vi "configuration UI.vi"() -> ()   [LabVIEW 2013, in "alarms module editor node.lvclass"]
uses:
  alarms module editor node.lvclass
  <vilib>/NI/Configuration Framework/Node/NodeRef.ctl
  <vilib>/NI/Configuration Framework/Node/NISE_CEF_Node.lvclass
  <vilib>/NI/AMC/Message Queue.ctl
  <vilib>/NI/AMC/Message.ctl
  <vilib>/NI/Tools/Keyed Array/KeyedArray.ctl
  <vilib>/NI/Configuration Framework/Node/UserEventRef.ctl
  <vilib>/NI/Configuration Framework/Controls/EventCluster.ctl
  <vilib>/NI/Configuration Framework/Node/StopEvent.ctl
  <vilib>/NI/Configuration Framework/Node/RefreshUIEvent.ctl
  <vilib>/NI/Configuration Framework/Node/CacheState.ctl
  <vilib>/NI/Configuration Framework/Node/NodeChangeEvent.ctl
  module/configuration/boolean operation.ctl
  module/configuration/compare type.ctl
  <vilib>/NI/Tag Bus/tag/Data Type.ctl
  alarms module editor node.lvclass/alarms module editor node.ctl
  <vilib>/NI/Configuration Framework/serializable configuration/NISE_CEF_serializable configuration.lvclass/NISE_CEF_serializable configuration.ctl
  <vilib>/NI/Tag Bus/tag/tag descriptor.lvclass/tag descriptor.ctl
  <vilib>/NI/Module Execution Interface/Engine Configuration/engine configuration.lvclass/engine configuration.ctl
  <vilib>/Utility/LVClass/Get LV Class Name.vi
  <vilib>/NI/Configuration Framework/error generator/NISE_error generator.vi
  <vilib>/NI/Tag Bus Module Framework/channel/TBM channel.lvclass
  <vilib>/NI/Module Execution Interface/Engine Configuration/engine configuration.lvclass
  <vilib>/NI/DCAF/Tag Editor Core/Configuration Editor/Classes/Module editor node/module editor node.lvclass
  <vilib>/NI/DCAF/Tag Editor Core/Configuration Editor/Classes/Engine Parent/Engine Parent Editor Node.lvclass
  <vilib>/NI/Configuration Framework/serializable configuration/NISE_CEF_serializable configuration.lvclass
  module/configuration/alarms module configuration.lvclass
  <vilib>/NI/Tag Bus/tag/tag descriptor.lvclass
  <vilib>/NI/Tools/Keyed Array/Tools_KeyedArray.lvlib
  <vilib>/NI/AMC/AMC.lvlib
  <vilib>/NI/Configuration Framework/NISE_CEF_TreeControl.lvlib
panel:
  in  "node change":T1
  in  "cache state":T2
  in  "refresh UI":T3
  in  "stop event":T4
  in  "Tab Control":enum32{"Alarm Configuration", "Alarm Table"}(tab)
  in  "data type":T5
  in  "Limit":dbl
  in  "comparison op":T6
  in  "Input Tag":string(combo)
  in  "Unlatch Tag":string(combo)
  in  "Output Tag":string(combo)
  in  "Remove compare":bool
  in  "Add compare":bool
  in  "Comparisons list":i32(listbox)
  out "alarm name":string
  in  "Alarms":i32(listbox)
  in  "Remove alarm":bool
  in  "Add alarm":bool
  in  "operation":T7
  in  "Full Alarms Table":i32(listbox)
  in  "user event":T8
  in  "main queue":T9
  in  "node ref":T10
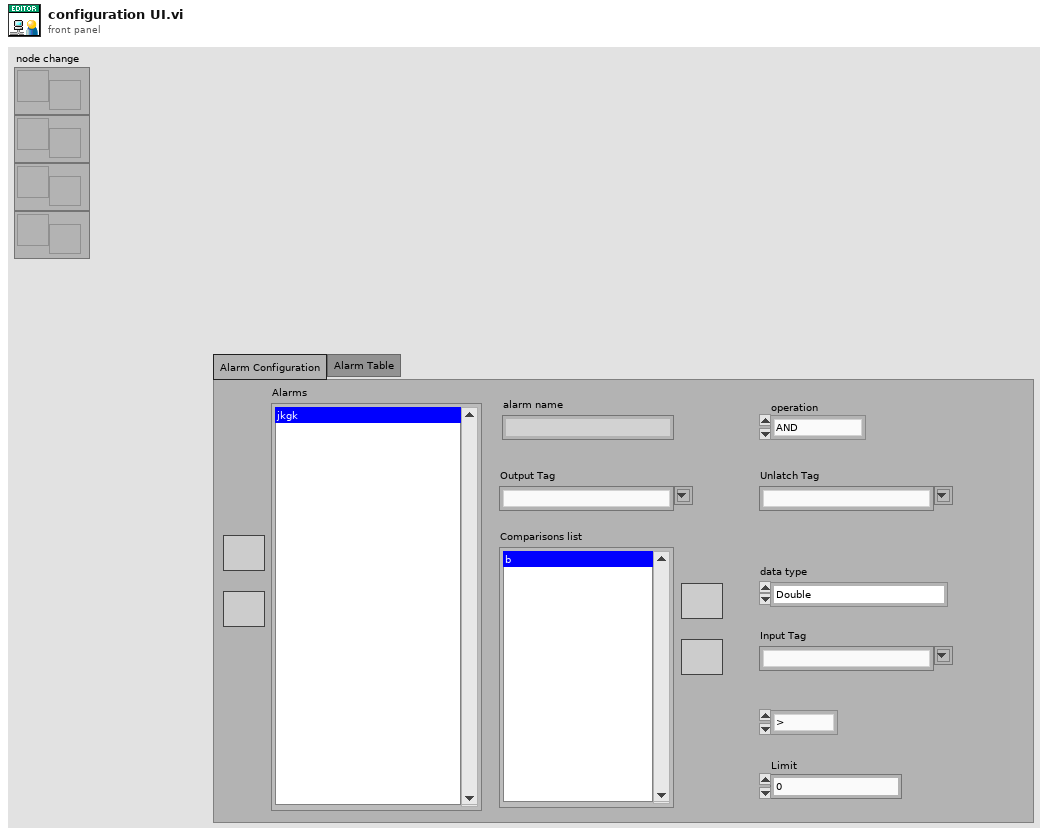
[diagram p1: front panel]
types:
  T1 = typedef "NISE_CEF_Node.lvclass/NodeChangeEvent.ctl" = refnum<user-event>
  T2 = typedef "NISE_CEF_Node.lvclass/CacheState.ctl" = refnum<user-event>
  T3 = typedef "NISE_CEF_Node.lvclass/RefreshUIEvent.ctl" = refnum<user-event>
  T4 = typedef "NISE_CEF_Node.lvclass/StopEvent.ctl" = refnum<user-event>
  T5 = typedef "tag bus.lvlib/tag descriptor.lvclass/Data Type.ctl" = enum16{"Double", "Single", "I64", "I32", "I16", "I8", "U64", "U32", "U16", "U8", "Boolean", "String", "Array of Double", "Array of Single", "Array of I64", "Array of I32", "Array of I16", "Array of I8", "Array of U64", "Array of U32", "Array of U16", "Array of U8", "Array of Boolean", "Array of String"}
  T6 = typedef "alarms module configuration.lvclass/compare type.ctl" = enum16{">", "<", ">=", "<=", "="}
  T7 = typedef "alarms module configuration.lvclass/boolean operation.ctl" = enum16{"AND", "OR"}
  T8 = typedef "NISE_CEF_Node.lvclass/UserEventRef.ctl" = refnum<user-event>
  T9 = typedef "AMC.lvlib/Message Queue.ctl" = refnum<queue>
  T10 = typedef "NISE_CEF_Node.lvclass/NodeRef.ctl" = refnum<data-value>
  T11 = enum8{"Enabled", "Disabled", "Disabled and Grayed Out"}
  T12 = typedef "alarms module configuration.lvclass/alarm configuration.ctl" = cluster{"alarm name":string, "comparisons":T13[], "unlatch":refnum<class "TBM channel.lvclass">, "output":refnum<class "TBM channel.lvclass">, "boolean op":T7}
  T13 = typedef "alarms module configuration.lvclass/alarm comparison.ctl" = cluster{"input channel":refnum<class "TBM channel.lvclass">, "limit":dbl, "comparison":T6}
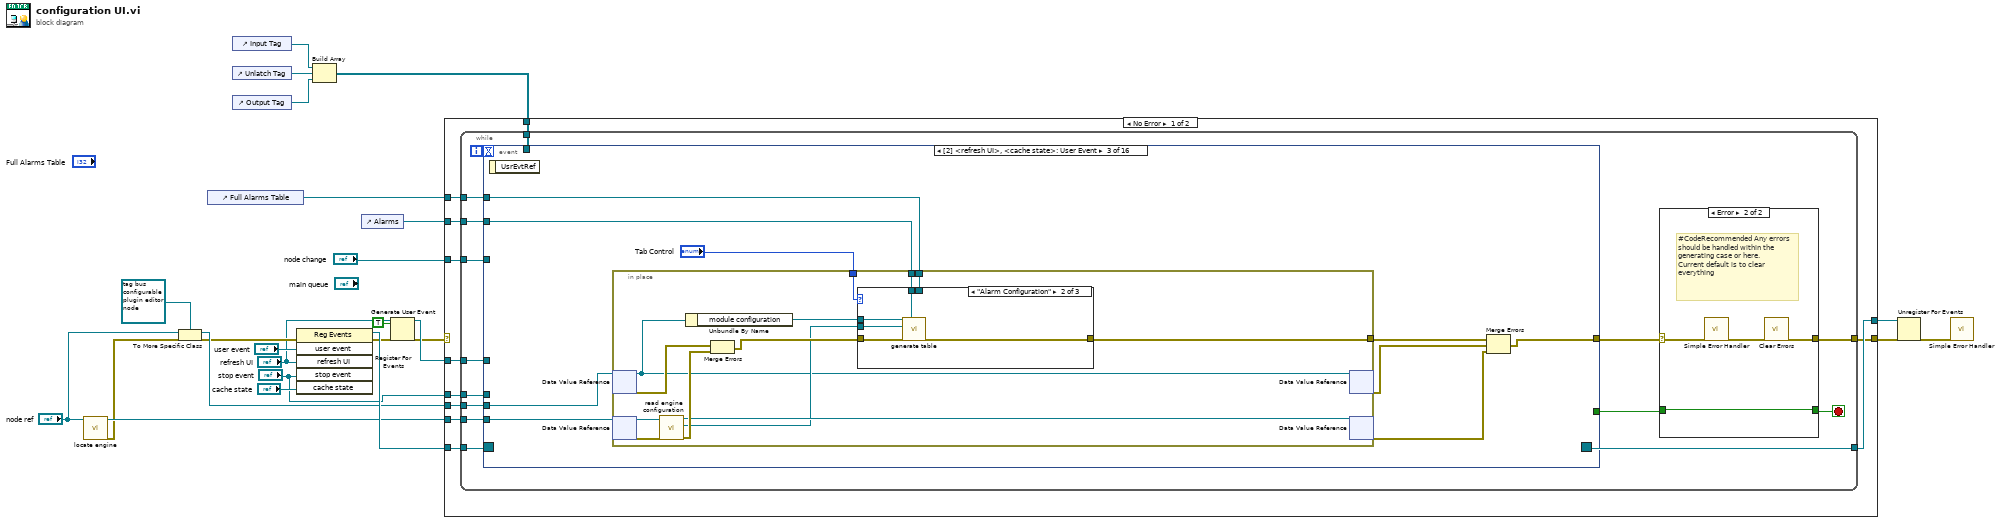
[diagram p0: block diagram]
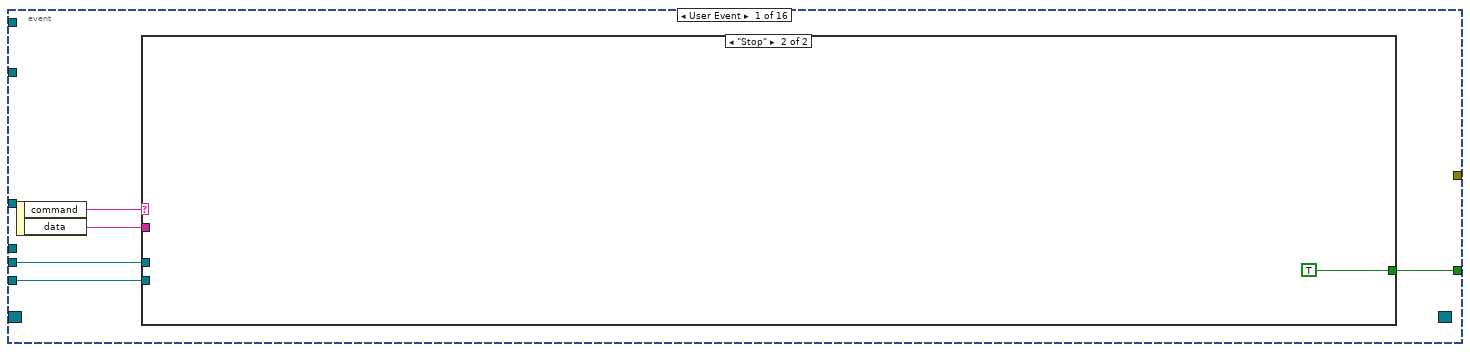
[diagram p3: hidden frame]
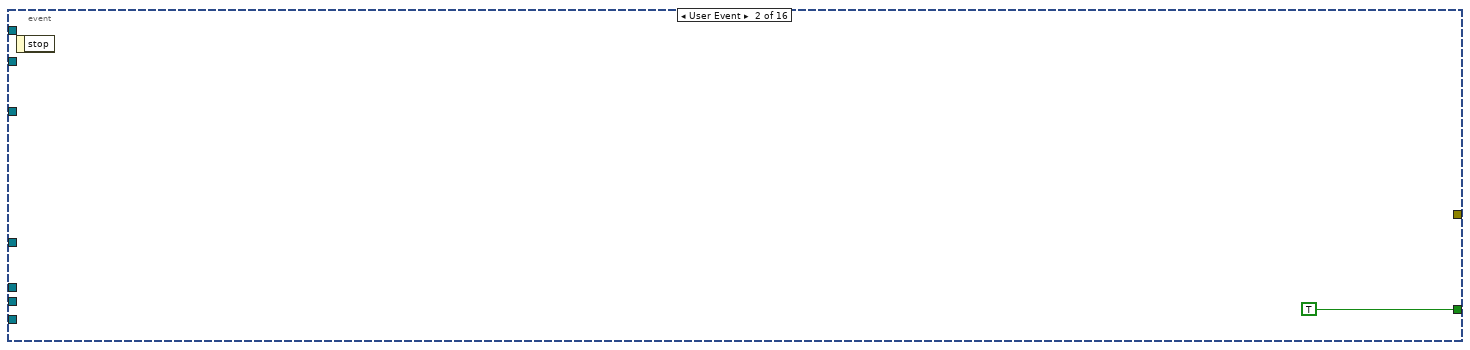
[diagram p5: hidden frame]
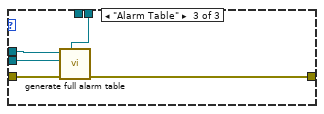
[diagram p7: hidden frame]
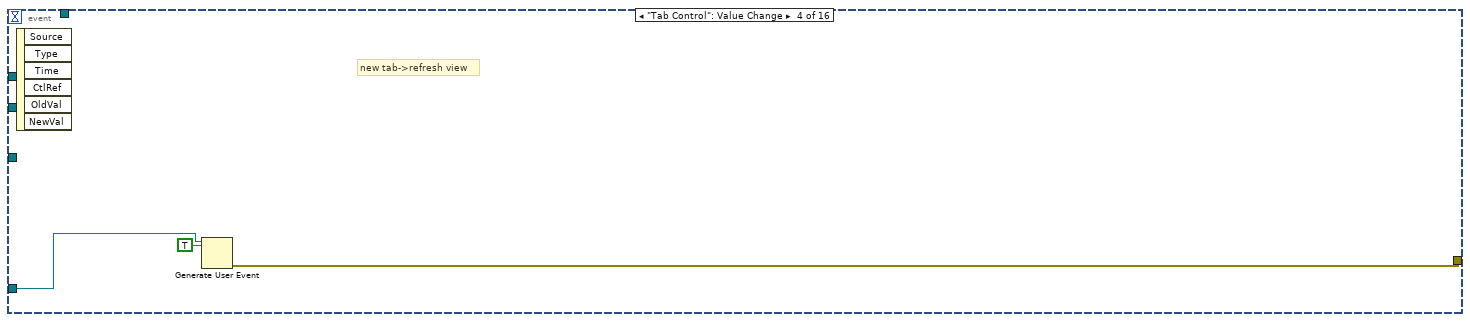
[diagram p8: hidden frame]
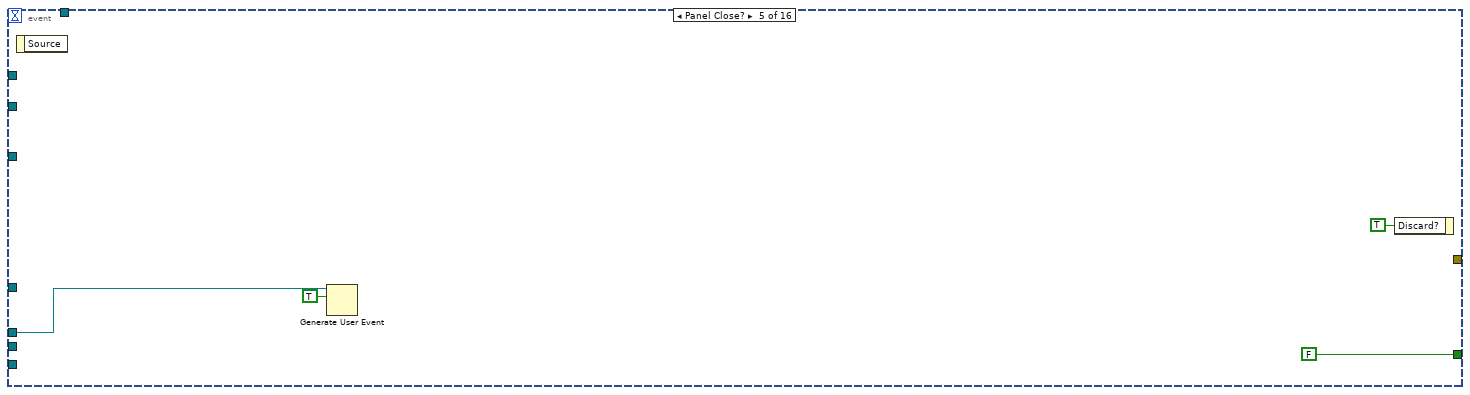
[diagram p9: hidden frame]
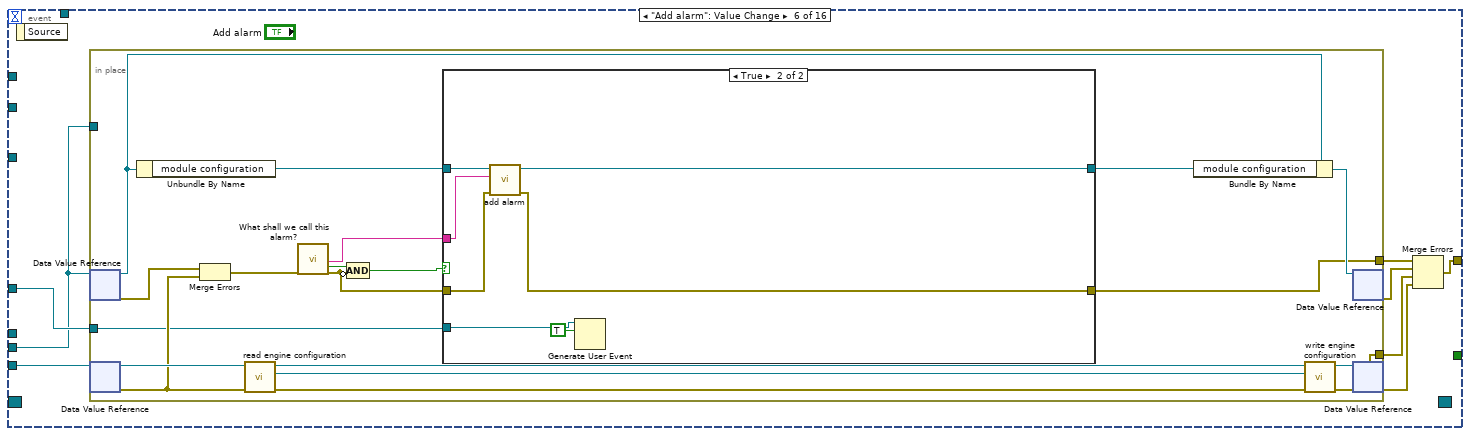
[diagram p10: hidden frame]
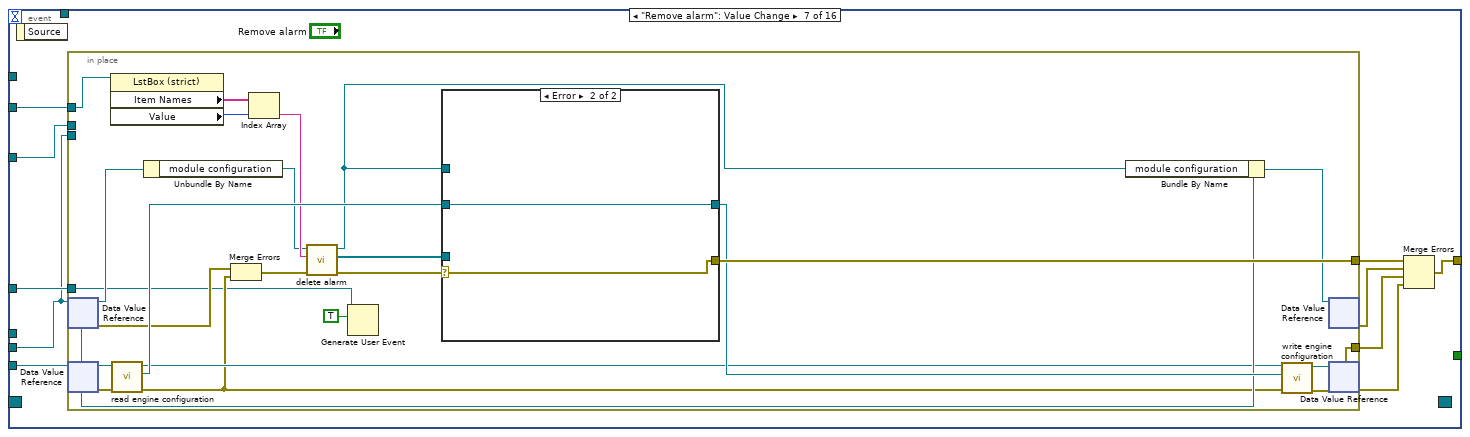
[diagram p12: hidden frame]
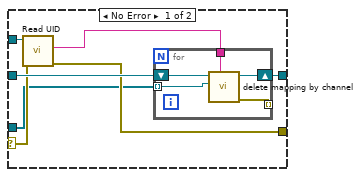
[diagram p13: hidden frame]
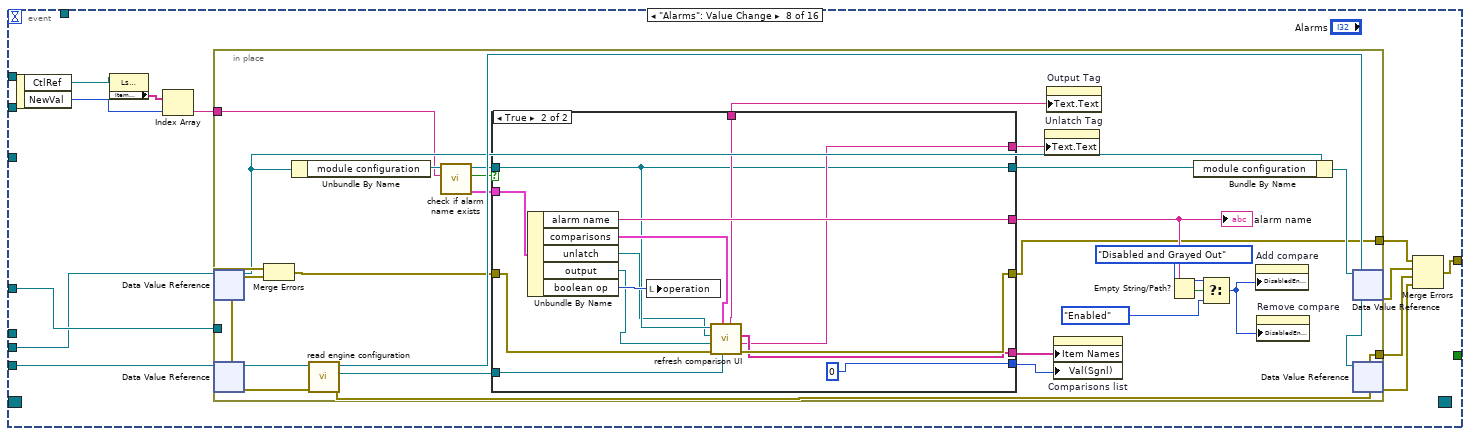
[diagram p14: hidden frame]
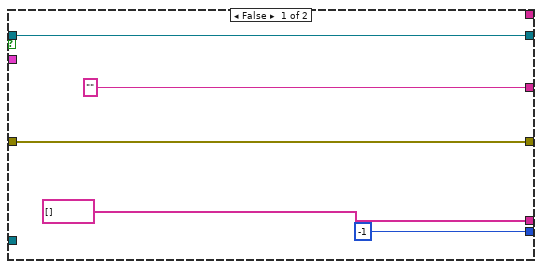
[diagram p15: hidden frame]
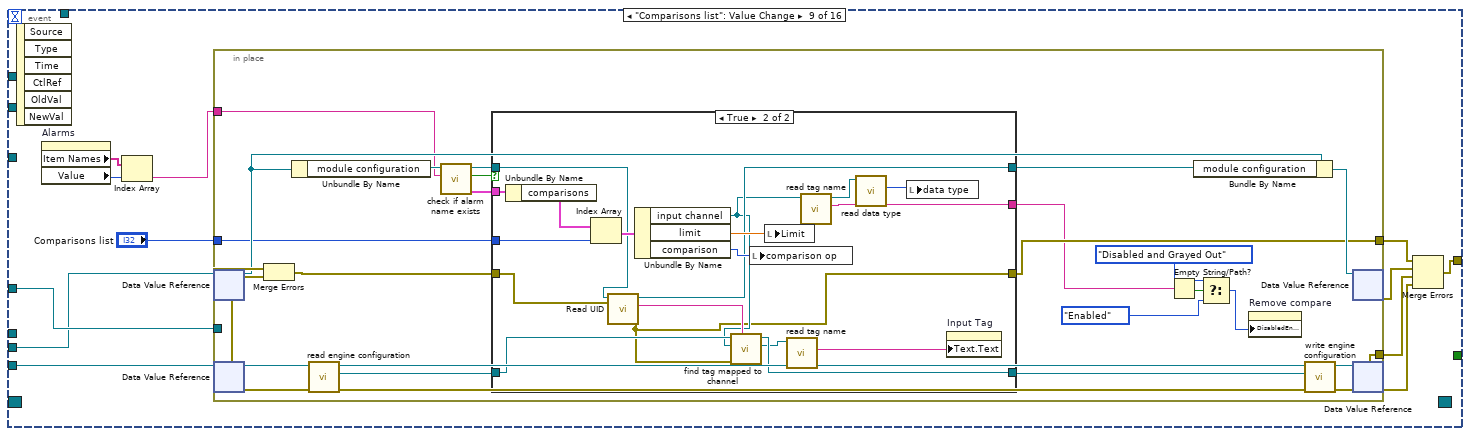
[diagram p16: hidden frame]
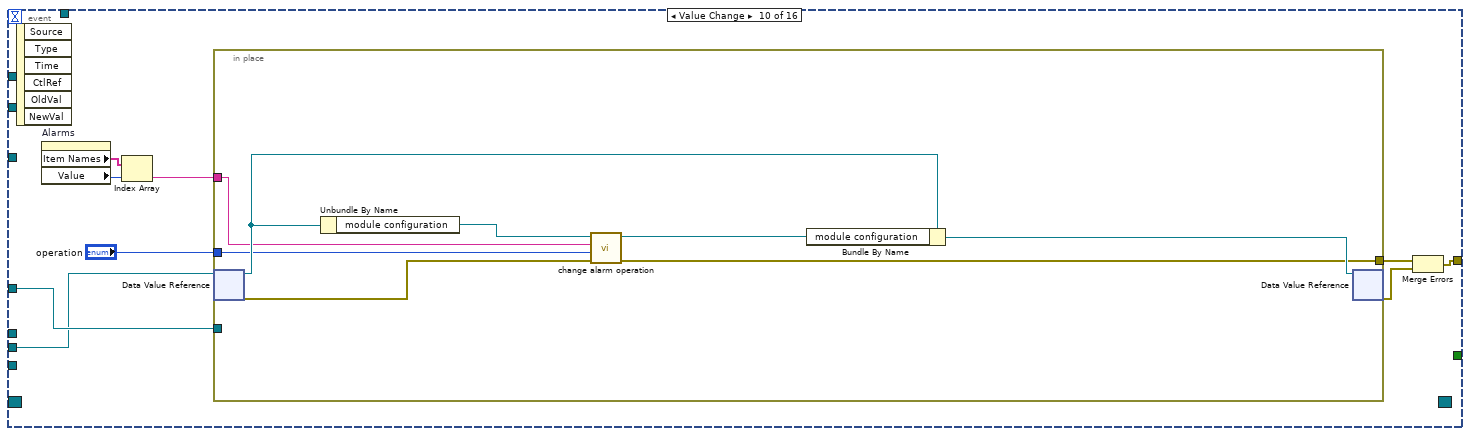
[diagram p18: hidden frame]
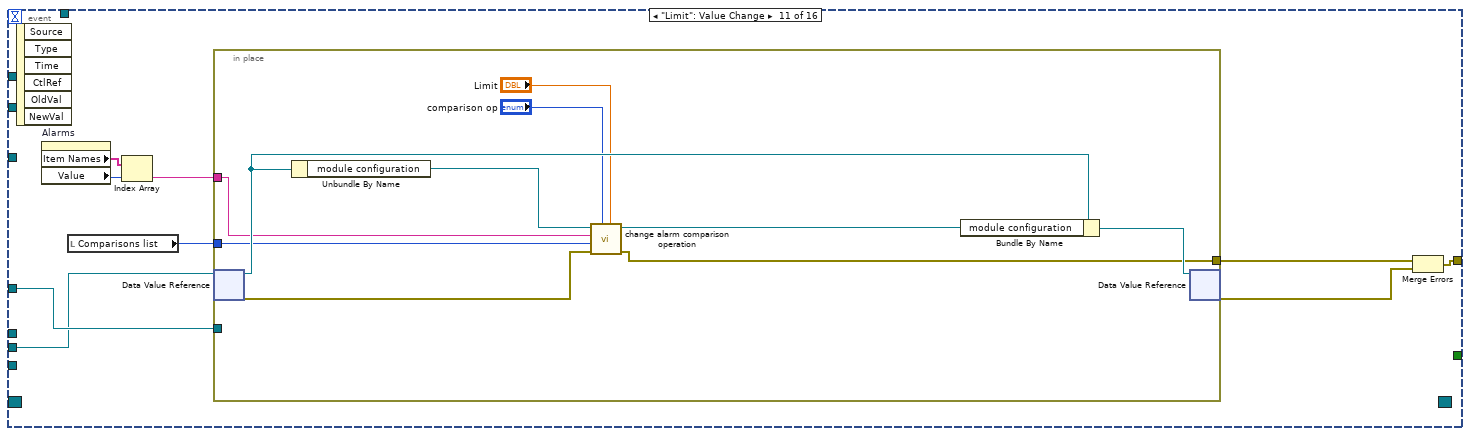
[diagram p19: hidden frame]
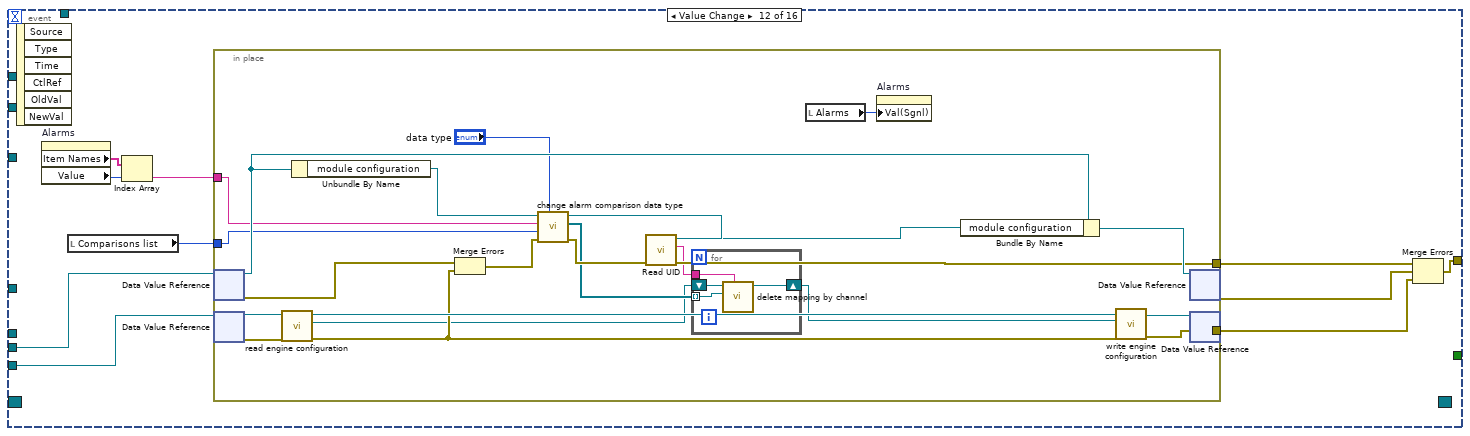
[diagram p20: hidden frame]
diagram:
  n1 = call <vilib>:"locate engine.vi"("component"="node ref") -> ("error out"=w14:errorcluster, "engine"=w20:refnum<data-value>)  [unwired: 9 in]
  n2 = To More Specific Class(target class=refnum<data-value> refnum ("data value reference"), reference="node ref", error in=w14) -> (specific class reference=w17:refnum<data-value>, error out=w16:errorcluster)
  n3 = control-ref of="Full Alarms Table"() -> (w5:refnum<vi>)
  n4 = control-ref of="Input Tag"() -> (w2:refnum<vi>)
  n5 = control-ref of="Unlatch Tag"() -> (w3:refnum<vi>)
  n6 = control-ref of="Output Tag"() -> (w4:refnum<vi>)
  n7 = register-events(error in=w16, "user event", "refresh UI", "stop event", "cache state") -> (reference out=w25:refnum<event-registration>, error out=w21:errorcluster)  [unwired: 1 in]
  n8 = Build Array(w2, w3, w4) -> (w1:refnum<vi>[])
  n9 = control-ref of="Alarms"() -> (w6:refnum<vi>)
  n10 = Generate User Event(user event="refresh UI", event data cluster=TRUE ("event data"), error in=w21) -> (user event out=w13:T3, error out=w8:errorcluster)  [unwired: 1 in]
  n11 = case shown="No Error" w8 {
    selector: w8 -> [_ w569]
    tunnel: w25 -> [w36 w568]
    tunnel: [w35 w568] -> w24
    tunnel: [w34 w569] -> w23
    tunnel: w20 -> [w33 _]
    tunnel: w17 -> [w32 _]
    tunnel: w13 -> [w31 _]
    tunnel: "node change" -> [w30 _]
    tunnel: "stop event" -> [w29 _]
    tunnel: w6 -> [w28 _]
    tunnel: w5 -> [w27 _]
    tunnel: w1 -> [w26 _]
    frame No Error {
      n12 = while {
        tunnel: w36 -> [w50]
        tunnel: [w49] -> w35
        tunnel: w32 -> [w45]
        tunnel: w33 -> [w44]
        tunnel: w31 -> [w43]
        tunnel: w30 -> [w41]
        tunnel: [w46] -> w34
        tunnel: w29 -> [w40]
        tunnel: w28 -> [w39]
        tunnel: w27 -> [w38]
        tunnel: w26 -> [w37]
        stop <- w48 stop-if-true
        n13 = event shown="[2] <refresh UI>, <cache state>: User Event" {
          selector: w50 -> [_ _ _ _ _ _ _ _ _ _ _ _ _ _ _ _]
          dyn-events: [_ _ _ _ _ _ _ _ _ _ _ _ _ _ _ _] -> w49
          timeout: _ -> [_ _ _ _ _ _ _ _ _ _ _ _ _ _ _ _]
          tunnel: [w61 TRUE _ _ FALSE _ _ _ _ _ _ _ _ _ _ _] -> w47
          tunnel: [_ _ w70 w97 _ w110 w146 w197 w253 w309 w326 w347 w385 w437 w481 w518] -> w42
          tunnel: w45 -> [w59 _ w72 _ _ w105 w141 w192 w248 w307 w324 w345 w387 w439 w483 w520]
          tunnel: w44 -> [w58 _ w71 _ _ w109 w147 w196 w252 _ _ w340 w380 _ w477 w513]
          tunnel: w43 -> [_ _ _ w98 _ w111 w148 w198 w254 w310 w327 _ _ _ _ _]
          tunnel: w41 -> [_ _ _ _ _ _ w142 _ _ _ _ _ _ _ _ _]
          tunnel: w40 -> [_ _ _ _ w101 _ _ _ _ _ _ _ _ _ _ _]
          tunnel: w39 -> [_ _ w65 _ _ _ w140 _ _ _ _ _ _ _ _ _]
          tunnel: w38 -> [_ _ w64 _ _ _ _ _ _ _ _ _ _ _ _ _]
          tunnel: w37 -> [_ _ _ _ _ _ _ _ _ _ _ _ w388 _ _ w521]
          event User Event {
            n14 = event-data() -> ("command"=w60:string, "data"=w57:string)  [unwired: 1 in]
            n15 = case shown="\"Stop\"" w60 {
              tunnel: [_ TRUE] -> w61
              tunnel: w59 -> [_ _]
              tunnel: w58 -> [_ _]
              tunnel: w57 -> [_ _]
              frame Default {
              }
              frame "Stop" {
              }
            }
          }
          event User Event {
            n16 = event-data() -> ()  [unwired: 1 in, 1 out]
          }
          event User Event {
            n17 = event-data() -> ()  [unwired: 1 in, 1 out]
            n18 = in-place {
              in-place-border: [w85] -> w69
              in-place-border: "Tab Control" -> [w75]
              in-place-border: w65 -> [w74]
              in-place-border: w64 -> [w73]
              n19 = in-place-dvr #1(w72) -> (w77:refnum<class "alarms module editor node.lvclass">, w83:errorcluster)
              n20 = in-place-dvr #2(w71) -> (w80:refnum<class "Engine Parent Editor Node.lvclass">, w82:errorcluster)
              n21 = call <vilib>:"read engine configuration.vi"("error in"=w82, "Engine Parent Editor Node in"=w80) -> ("error out"=w81:errorcluster, "engine configuration"=w78:refnum<class "engine configuration.lvclass">, "Engine Parent Editor Node out"=w79:refnum<class "Engine Parent Editor Node.lvclass">)  [unwired: 7 in]
              n22 = Unbundle By Name(w77) -> ("module configuration"=w76:refnum<class "alarms module configuration.lvclass">)
              n23 = Merge Errors(w83, w81) -> (w84:errorcluster)
              n24 = case shown="\"Alarm Configuration\"" w75 {
                tunnel: [w86 w91 w95] -> w85
                tunnel: w84 -> [w86 w90 w96]
                tunnel: w78 -> [_ w89 w92]
                tunnel: w76 -> [_ w88 w93]
                tunnel: w74 -> [_ w87 _]
                tunnel: w73 -> [_ _ w94]
                frame Default {
                }
                frame "Alarm Configuration" {
                  n25 = call "generate table.vi"("Alarms list"=w87, "error in"=w90, "engine configuration"=w89, "tag bus configurable plugin module configuration"=w88) -> ("error out"=w91:errorcluster)  [unwired: 7 in]
                }
                frame "Alarm Table" {
                  n26 = call "generate full alarm table.vi"("Full Alarms Table"=w94, "error in"=w96, "engine configuration"=w92, "tag bus configurable plugin module configuration"=w93) -> ("error out"=w95:errorcluster)  [unwired: 7 in]
                }
              }
              n27 = in-place-dvr #1(w77) -> (w68:errorcluster)  [unwired: 1 out]
              n28 = in-place-dvr #2(w79) -> (w67:errorcluster)  [unwired: 1 out]
            }
            n29 = Merge Errors(w69, w68, w67) -> (w70:errorcluster)
          }
          event "Tab Control": Value Change {
            # "new tab->refresh view"
            n30 = event-data() -> ()  [unwired: 1 in, 6 out]
            n31 = Generate User Event(user event=w98, event data cluster=TRUE ("event data")) -> (error out=w97:errorcluster)  [unwired: 2 in, 1 out]
          }
          event Panel Close? {
            n32 = event-data() -> ()  [unwired: 1 in, 1 out]
            n33 = Generate User Event(user event=w101, event data cluster=TRUE ("event data")) -> ()  [unwired: 2 in, 2 out]
            n34 = event-data("Discard?"=TRUE) -> ()  [unwired: 1 in, 1 out]
          }
          event "Add alarm": Value Change {
            n35 = event-data() -> ()  [unwired: 1 in, 1 out]
            n36 = in-place {
              in-place-border: w111 -> [w112]
              in-place-border: [w127] -> w107
              in-place-border: w105 -> [_]
              in-place-border: [w115] -> w104
              n37 = in-place-dvr #3(w105) -> (w123:refnum<class "alarms module editor node.lvclass">, w124:errorcluster)
              n38 = in-place-dvr #4(w109) -> (w130:refnum<class "Engine Parent Editor Node.lvclass">, w129:errorcluster)
              n39 = Unbundle By Name(w123) -> ("module configuration"=w116:refnum<class "alarms module configuration.lvclass">)
              n40 = Merge Errors(w124, w129) -> (w121:errorcluster)
              n41 = call <vilib>:"read engine configuration.vi"("error in"=w129, "Engine Parent Editor Node in"=w130) -> ("error out"=w125:errorcluster, "engine configuration"=w113:refnum<class "engine configuration.lvclass">, "Engine Parent Editor Node out"=w126:refnum<class "Engine Parent Editor Node.lvclass">)  [unwired: 7 in]
              n42 = call "What shall we call this alarm?"("error in (no error)"=w121) -> ("Alarm Name"=w114:string, "OK"=w120:bool, "error out"=w119:errorcluster)  [unwired: 16 in]
              n43 = Compound Arithmetic op=AND(w120, invert w119) -> (w118:bool)
              n44 = case shown="True" w118 {
                tunnel: w119 -> [w131 w138]
                tunnel: [w132 w137] -> w117
                tunnel: w116 -> [w132 w139]
                tunnel: [w131 w135] -> w115
                tunnel: w114 -> [_ w136]
                tunnel: w112 -> [_ w134]
                frame False {
                }
                frame True {
                  n45 = call "add alarm.vi"("error in"=w138, "alarm name"=w136, "alarms module configuration in"=w139) -> ("error out"=w135:errorcluster, "alarms module configuration out"=w137:refnum<class "alarms module configuration.lvclass">)  [unwired: 6 in, 1 out]
                  n46 = Generate User Event(user event=w134, event data cluster=TRUE ("event data")) -> ()  [unwired: 2 in, 2 out]
                }
              }
              n47 = Bundle By Name(cluster=w123, "module configuration"=w117) -> (w122:refnum<class "alarms module editor node.lvclass">)
              n48 = call <vilib>:"write engine configuration.vi"("error in"=w125, "engine configuration"=w113, "Engine Parent Editor Node in"=w126) -> ("error out"=w127:errorcluster, "Engine Parent Editor Node out"=w128:refnum<class "Engine Parent Editor Node.lvclass">)  [unwired: 7 in]
              n49 = in-place-dvr #3(w122) -> (w106:errorcluster)  [unwired: 1 out]
              n50 = in-place-dvr #4(w128) -> (w108:errorcluster)  [unwired: 1 out]
            }
            n51 = Merge Errors(w104, w106, w107, w108) -> (w110:errorcluster)
          }
          event "Remove alarm": Value Change {
            n52 = event-data() -> ()  [unwired: 1 in, 1 out]
            n53 = in-place {
              in-place-border: [w172] -> w149
              in-place-border: w148 -> [w152]
              in-place-border: [w170] -> w143
              in-place-border: w142 -> [_]
              in-place-border: w141 -> [_]
              in-place-border: w140 -> [w160]
              n54 = in-place-dvr #5(w141) -> (w165:refnum<class "alarms module editor node.lvclass">, w161:errorcluster)
              n55 = in-place-dvr #6(w147) -> (w167:refnum<class "Engine Parent Editor Node.lvclass">, w166:errorcluster)
              n56 = property class="LstBox (strict)"(reference=w160) -> ("Item Names"=w158:string[], "Value"=w159:i32)  [unwired: 1 in, 2 out]
              n57 = call <vilib>:"read engine configuration.vi"("error in"=w166, "Engine Parent Editor Node in"=w167) -> ("error out"=w162:errorcluster, "engine configuration"=w164:refnum<class "engine configuration.lvclass">, "Engine Parent Editor Node out"=w163:refnum<class "Engine Parent Editor Node.lvclass">)  [unwired: 7 in]
              n58 = Unbundle By Name(w165) -> ("module configuration"=w155:refnum<class "alarms module configuration.lvclass">)
              n59 = Merge Errors(w161, w162) -> (w157:errorcluster)
              n60 = Index Array(array=w158, index=w159) -> (element=w156:string)
              n61 = call "delete alarm.vi"("error in"=w157, "alarm name"=w156, "alarms module configuration in"=w155) -> ("error out"=w154:errorcluster, "deleted channels"=w151:refnum<class "TBM channel.lvclass">[], "alarms module configuration out"=w150:refnum<class "alarms module configuration.lvclass">)  [unwired: 6 in]
              n62 = Generate User Event(user event=w152, event data cluster=TRUE ("event data")) -> ()  [unwired: 2 in, 2 out]
              n63 = case shown="Error" w154 {
                selector: w154 -> [w175 w185]
                tunnel: [w174 w185] -> w172
                tunnel: w150 -> [w177 _]
                tunnel: w164 -> [w179 w186]
                tunnel: [w178 w186] -> w168
                tunnel: w151 -> [w173 _]
                frame No Error {
                  n64 = call <vilib>:"Read UID.vi"("error in"=w175, "configuration in"=w177) -> ("error out"=w174:errorcluster, "instance id"=w176:string)  [unwired: 7 in, 1 out]
                  n65 = for {
                    tunnel: w176 -> [w182]
                    shift-right: [w183] -> w178
                    shift-left: w179 -> [w184]
                    tunnel: [w181] -> _ mode=indexing
                    tunnel: w173 -> [w180] mode=indexing
                    n66 = call <vilib>:"delete mapping by channel.vi"("owner ID"=w182, "channel"=w180, "engine configuration in"=w184) -> ("error out"=w181:errorcluster, "engine configuration out"=w183:refnum<class "engine configuration.lvclass">)  [unwired: 7 in]
                  }
                }
                frame Error {
                }
              }
              n67 = Bundle By Name(cluster=w165, "module configuration"=w150) -> (w169:refnum<class "alarms module editor node.lvclass">)
              n68 = call <vilib>:"write engine configuration.vi"("error in"=w162, "engine configuration"=w168, "Engine Parent Editor Node in"=w163) -> ("error out"=w170:errorcluster, "Engine Parent Editor Node out"=w171:refnum<class "Engine Parent Editor Node.lvclass">)  [unwired: 7 in]
              n69 = in-place-dvr #5(w169) -> (w144:errorcluster)  [unwired: 1 out]
              n70 = in-place-dvr #6(w171) -> (w145:errorcluster)  [unwired: 1 out]
            }
            n71 = Merge Errors(w149, w144, w143, w145) -> (w146:errorcluster)
          }
          event "Alarms": Value Change {
            n72 = event-data() -> ("CtlRef"=w190:refnum<vi>, "NewVal"=w189:i32)  [unwired: 1 in]
            n73 = property class="LstBox (strict)"(reference=w190) -> ("Item Names"=w191:string[])  [unwired: 1 in, 2 out]
            n74 = Index Array(array=w191, index=w189) -> (element=w188:string)
            n75 = in-place {
              in-place-border: w198 -> [_]
              in-place-border: [w220] -> w194
              in-place-border: w188 -> [w215]
              in-place-border: [w204] -> w187
              n76 = in-place-dvr #7(w192) -> (w218:refnum<class "alarms module editor node.lvclass">, w219:errorcluster)
              n77 = in-place-dvr #8(w196) -> (w223:refnum<class "Engine Parent Editor Node.lvclass">, w222:errorcluster)
              n78 = Merge Errors(w219, w222) -> (w205:errorcluster)
              n79 = Unbundle By Name(w218) -> ("module configuration"=w216:refnum<class "alarms module configuration.lvclass">)
              n80 = call <vilib>:"read engine configuration.vi"("error in"=w222, "Engine Parent Editor Node in"=w223) -> ("error out"=w220:errorcluster, "engine configuration"=w211:refnum<class "engine configuration.lvclass">, "Engine Parent Editor Node out"=w221:refnum<class "Engine Parent Editor Node.lvclass">)  [unwired: 7 in]
              n81 = call "check if alarm name exists.vi"("name to locate"=w215, "alarms module configuration in"=w216) -> ("alarm config"=w210:T12, "found?"=w214:bool, "alarms module configuration out"=w213:refnum<class "alarms module configuration.lvclass">)  [unwired: 6 in, 1 out]
              n82 = case shown="True" w214 {
                tunnel: w213 -> [w228 w232]
                tunnel: [w228 w232] -> w212
                tunnel: w211 -> [_ w229]
                tunnel: w210 -> [_ w242]
                tunnel: ["" ("alarm name") w241] -> w209
                tunnel: w205 -> [w227 w239]
                tunnel: [w227 w238] -> w204
                tunnel: [string[] [] ("Item Names") w236] -> w203
                tunnel: [-1 ("Value (Signaling)") 0 ("Value (Signaling)")] -> w202
                tunnel: [_ w234] -> w201
                tunnel: [_ w233] -> w200
                frame False {
                }
                frame True {
                  n83 = Unbundle By Name(w242) -> ("alarm name"=w241:string, "comparisons"=w237:T13[], "unlatch"=w231:refnum<class "TBM channel.lvclass">, "output"=w230:refnum<class "TBM channel.lvclass">, "boolean op"=w240:T7)
                  n84 = local write "operation"(w240) -> ()
                  n85 = call "refresh comparison UI.vi"("engine configuration"=w229, "comparisons"=w237, "error in\\"=w239, "output"=w230, "unlatch"=w231, "alarms module configuration in"=w232) -> ("error out"=w238:errorcluster, "unlatch tag"=w234:string, "Item Names"=w236:string[], "output tag"=w233:string)  [unwired: 2 in]
                }
              }
              "alarm name" <- w209
              n86 = property on="Unlatch Tag" class="CmbBox"("Text.Text"=w201) -> ()  [unwired: 2 in, 2 out]
              n87 = property on="Output Tag" class="CmbBox"("Text.Text"=w200) -> ()  [unwired: 2 in, 2 out]
              n88 = property on="Comparisons list" class="LstBox (strict)"("Item Names"=w203, "Val(Sgnl)"=w202) -> ()  [unwired: 2 in, 2 out]
              n89 = Empty String/Path?(string/path=w209) -> (empty?=w208:bool)
              n90 = Bundle By Name(cluster=w218, "module configuration"=w212) -> (w217:refnum<class "alarms module editor node.lvclass">)
              n91 = Select(t=T11."Disabled and Grayed Out" ("Disabled"), s=w208, f=T11."Enabled" ("Disabled")) -> (s? t:f=w199:T11)
              n92 = property on="Add compare" class="Bool"("DisabledEnum"=w199) -> ()  [unwired: 2 in, 2 out]
              n93 = property on="Remove compare" class="Bool"("DisabledEnum"=w199) -> ()  [unwired: 2 in, 2 out]
              n94 = in-place-dvr #7(w217) -> (w193:errorcluster)  [unwired: 1 out]
              n95 = in-place-dvr #8(w221) -> (w195:errorcluster)  [unwired: 1 out]
            }
            n96 = Merge Errors(w187, w193, w194, w195) -> (w197:errorcluster)
          }
          event "Comparisons list": Value Change {
            n97 = event-data() -> ()  [unwired: 1 in, 6 out]
            n98 = property on="Alarms" class="LstBox (strict)"() -> ("Item Names"=w246:string[], "Value"=w245:i32)  [unwired: 2 in, 2 out]
            n99 = Index Array(array=w246, index=w245) -> (element=w244:string)
            n100 = in-place {
              in-place-border: w254 -> [_]
              in-place-border: [w276] -> w250
              in-place-border: w244 -> [w269]
              in-place-border: [w257] -> w247
              in-place-border: "Comparisons list" -> [w256]
              n101 = in-place-dvr #9(w248) -> (w272:refnum<class "alarms module editor node.lvclass">, w273:errorcluster)
              n102 = in-place-dvr #10(w252) -> (w279:refnum<class "Engine Parent Editor Node.lvclass">, w278:errorcluster)
              n103 = Merge Errors(w273, w278) -> (w258:errorcluster)
              n104 = Unbundle By Name(w272) -> ("module configuration"=w270:refnum<class "alarms module configuration.lvclass">)
              n105 = call <vilib>:"read engine configuration.vi"("error in"=w278, "Engine Parent Editor Node in"=w279) -> ("error out"=w274:errorcluster, "engine configuration"=w265:refnum<class "engine configuration.lvclass">, "Engine Parent Editor Node out"=w275:refnum<class "Engine Parent Editor Node.lvclass">)  [unwired: 7 in]
              n106 = call "check if alarm name exists.vi"("name to locate"=w269, "alarms module configuration in"=w270) -> ("alarm config"=w263:T12, "found?"=w268:bool, "alarms module configuration out"=w267:refnum<class "alarms module configuration.lvclass">)  [unwired: 6 in, 1 out]
              n107 = case shown="True" w268 {
                tunnel: w267 -> [w282 w291]
                tunnel: [w282 w290] -> w266
                tunnel: w265 -> [w281 w293]
                tunnel: [w281 w292] -> w264
                tunnel: w263 -> [_ w301]
                tunnel: w258 -> [w280 w300]
                tunnel: [w280 w287] -> w257
                tunnel: w256 -> [_ w298]
                tunnel: [_ w296] -> w255
                frame False {
                }
                frame True {
                  n108 = Unbundle By Name(w301) -> ("comparisons"=w299:T13[])
                  n109 = Index Array(array=w299, index=w298) -> (element=w297:T13)
                  n110 = call <vilib>:"Read UID.vi"("error in"=w300, "configuration in"=w291) -> ("error out"=w287:errorcluster, "instance id"=w289:string, "configuration out"=w290:refnum<class "alarms module configuration.lvclass">)  [unwired: 7 in]
                  n111 = Unbundle By Name(w297) -> ("input channel"=w288:refnum<class "TBM channel.lvclass">, "limit"=w295:dbl, "comparison"=w294:T6)
                  n112 = call <vilib>:"find tag mapped to channel.vi"("owner"=w289, "error in"=w287, "channel"=w288, "engine configuration in"=w293) -> ("tag"=w286:refnum<class "tag descriptor.lvclass">, "engine configuration out"=w292:refnum<class "engine configuration.lvclass">)  [unwired: 5 in, 1 out]
                  n113 = local write "comparison op"(w294) -> ()
                  n114 = local write "Limit"(w295) -> ()
                  n115 = call <vilib>:"read tag name.vi"("system tag in"=w286) -> ("name"=w285:string)  [unwired: 8 in, 2 out]
                  n116 = call <vilib>:"read tag name.vi"("system tag in"=w288) -> ("name"=w296:string, "system tag out"=w284:refnum<class "TBM channel.lvclass">)  [unwired: 8 in, 1 out]
                  n117 = call <vilib>:"read data type.vi"("system tag in"=w284) -> ("data type"=w283:T5)  [unwired: 8 in, 2 out]
                  n118 = local write "data type"(w283) -> ()
                  n119 = property on="Input Tag" class="CmbBox"("Text.Text"=w285) -> ()  [unwired: 2 in, 2 out]
                }
              }
              n120 = Empty String/Path?(string/path=w255) -> (empty?=w262:bool)
              n121 = Bundle By Name(cluster=w272, "module configuration"=w266) -> (w271:refnum<class "alarms module editor node.lvclass">)
              n122 = Select(t=T11."Disabled and Grayed Out" ("Disabled"), s=w262, f=T11."Enabled" ("Disabled")) -> (s? t:f=w259:T11)
              n123 = property on="Remove compare" class="Bool"("DisabledEnum"=w259) -> ()  [unwired: 2 in, 2 out]
              n124 = call <vilib>:"write engine configuration.vi"("error in"=w274, "engine configuration"=w264, "Engine Parent Editor Node in"=w275) -> ("error out"=w276:errorcluster, "Engine Parent Editor Node out"=w277:refnum<class "Engine Parent Editor Node.lvclass">)  [unwired: 7 in]
              n125 = in-place-dvr #9(w271) -> (w249:errorcluster)  [unwired: 1 out]
              n126 = in-place-dvr #10(w277) -> (w251:errorcluster)  [unwired: 1 out]
            }
            n127 = Merge Errors(w247, w249, w250, w251) -> (w253:errorcluster)
          }
          event Value Change {
            n128 = event-data() -> ()  [unwired: 1 in, 6 out]
            n129 = property on="Alarms" class="LstBox (strict)"() -> ("Item Names"=w306:string[], "Value"=w305:i32)  [unwired: 2 in, 2 out]
            n130 = Index Array(array=w306, index=w305) -> (element=w304:string)
            n131 = in-place {
              in-place-border: w310 -> [_]
              in-place-border: w304 -> [w314]
              in-place-border: "operation" -> [w313]
              in-place-border: [w311] -> w302
              n132 = in-place-dvr #11(w307) -> (w318:refnum<class "alarms module editor node.lvclass">, w312:errorcluster)
              n133 = Unbundle By Name(w318) -> ("module configuration"=w316:refnum<class "alarms module configuration.lvclass">)
              n134 = call "change alarm operation.vi"("error in"=w312, "boolean op"=w313, "alarm name"=w314, "alarms module configuration in"=w316) -> ("error out"=w311:errorcluster, "alarms module configuration out"=w315:refnum<class "alarms module configuration.lvclass">)  [unwired: 6 in]
              n135 = Bundle By Name(cluster=w318, "module configuration"=w315) -> (w317:refnum<class "alarms module editor node.lvclass">)
              n136 = in-place-dvr #11(w317) -> (w308:errorcluster)  [unwired: 1 out]
            }
            n137 = Merge Errors(w302, w308) -> (w309:errorcluster)
          }
          event "Limit": Value Change {
            n138 = event-data() -> ()  [unwired: 1 in, 6 out]
            n139 = property on="Alarms" class="LstBox (strict)"() -> ("Item Names"=w323:string[], "Value"=w322:i32)  [unwired: 2 in, 2 out]
            n140 = local read "Comparisons list"() -> (w319:i32)
            n141 = Index Array(array=w323, index=w322) -> (element=w321:string)
            n142 = in-place {
              in-place-border: w327 -> [_]
              in-place-border: w321 -> [w333]
              in-place-border: [w331] -> w320
              in-place-border: w319 -> [w328]
              n143 = in-place-dvr #12(w324) -> (w337:refnum<class "alarms module editor node.lvclass">, w332:errorcluster)
              n144 = Unbundle By Name(w337) -> ("module configuration"=w335:refnum<class "alarms module configuration.lvclass">)
              n145 = call "change alarm comparison operation.vi"("Limit"="Limit", "comparison"="comparison op", "error in"=w332, "compare index"=w328, "alarm name"=w333, "alarms module configuration in"=w335) -> ("error out"=w331:errorcluster, "alarms module configuration out"=w334:refnum<class "alarms module configuration.lvclass">)  [unwired: 4 in]
              n146 = Bundle By Name(cluster=w337, "module configuration"=w334) -> (w336:refnum<class "alarms module editor node.lvclass">)
              n147 = in-place-dvr #12(w336) -> (w325:errorcluster)  [unwired: 1 out]
            }
            n148 = Merge Errors(w320, w325) -> (w326:errorcluster)
          }
          event Value Change {
            n149 = event-data() -> ()  [unwired: 1 in, 6 out]
            n150 = property on="Alarms" class="LstBox (strict)"() -> ("Item Names"=w344:string[], "Value"=w343:i32)  [unwired: 2 in, 2 out]
            n151 = local read "Comparisons list"() -> (w341:i32)
            n152 = Index Array(array=w344, index=w343) -> (element=w342:string)
            n153 = in-place {
              in-place-border: w342 -> [w366]
              in-place-border: w341 -> [w365]
              in-place-border: [w363] -> w339
              in-place-border: [w354] -> w338
              n154 = in-place-dvr #13(w345) -> (w370:refnum<class "alarms module editor node.lvclass">, w359:errorcluster)
              n155 = in-place-dvr #14(w340) -> (w361:refnum<class "Engine Parent Editor Node.lvclass">, w362:errorcluster)
              n156 = call <vilib>:"read engine configuration.vi"("error in"=w362, "Engine Parent Editor Node in"=w361) -> ("error out"=w358:errorcluster, "engine configuration"=w350:refnum<class "engine configuration.lvclass">, "Engine Parent Editor Node out"=w360:refnum<class "Engine Parent Editor Node.lvclass">)  [unwired: 7 in]
              n157 = Unbundle By Name(w370) -> ("module configuration"=w368:refnum<class "alarms module configuration.lvclass">)
              n158 = Merge Errors(w359, w358) -> (w357:errorcluster)
              n159 = call "change alarm comparison data type.vi"("data type"="data type", "error in"=w357, "compare index"=w365, "alarm name"=w366, "alarms module configuration in"=w368) -> ("error out"=w356:errorcluster, "changed channel"=w355:refnum<class "TBM channel.lvclass">[], "alarms module configuration out"=w353:refnum<class "alarms module configuration.lvclass">)  [unwired: 4 in]
              n160 = call <vilib>:"Read UID.vi"("error in"=w356, "configuration in"=w353) -> ("error out"=w354:errorcluster, "instance id"=w351:string, "configuration out"=w352:refnum<class "alarms module configuration.lvclass">)  [unwired: 7 in]
              n161 = for {
                shift-right: [w374] -> w349
                shift-left: w350 -> [w373]
                tunnel: w355 -> [w372] mode=indexing
                tunnel: w351 -> [w371]
                n162 = call <vilib>:"delete mapping by channel.vi"("owner ID"=w371, "channel"=w372, "engine configuration in"=w373) -> ("engine configuration out"=w374:refnum<class "engine configuration.lvclass">)  [unwired: 7 in, 1 out]
              }
              n163 = local read "Alarms"() -> (w348:i32)
              n164 = property on="Alarms" class="LstBox (strict)"("Val(Sgnl)"=w348) -> ()  [unwired: 2 in, 2 out]
              n165 = Bundle By Name(cluster=w370, "module configuration"=w352) -> (w369:refnum<class "alarms module editor node.lvclass">)
              n166 = call <vilib>:"write engine configuration.vi"("error in"=w358, "engine configuration"=w349, "Engine Parent Editor Node in"=w360) -> ("error out"=w363:errorcluster, "Engine Parent Editor Node out"=w364:refnum<class "Engine Parent Editor Node.lvclass">)  [unwired: 7 in]
              n167 = in-place-dvr #13(w369) -> (w346:errorcluster)  [unwired: 1 out]
              n168 = in-place-dvr #14(w364) -> ()  [unwired: 2 out]
            }
            n169 = Merge Errors(w338, w346, w339) -> (w347:errorcluster)
          }
          event "Output Tag", "Unlatch Tag", "Input Tag": Mouse Down? {
            n170 = event-data() -> ("CtlRef"=w376:refnum<vi>)  [unwired: 1 in, 4 out]
            n171 = property on="Alarms" class="LstBox (strict)"() -> ("Item Names"=w384:string[], "Value"=w383:i32)  [unwired: 2 in, 2 out]
            n172 = local read "Comparisons list"() -> (w378:i32)
            n173 = Search 1D Array(1D array=w388, element=w376) -> (index of element=w381:i32)  [unwired: 1 in]
            n174 = Index Array(array=w384, index=w383) -> (element=w382:string)
            n175 = in-place {
              in-place-border: w382 -> [w406]
              in-place-border: w381 -> [w403]
              in-place-border: w378 -> [w399]
              in-place-border: [w397] -> w377
              in-place-border: w376 -> [w396]
              n176 = in-place-dvr #15(w387) -> (w408:refnum<class "alarms module editor node.lvclass">)  [unwired: 1 out]
              n177 = in-place-dvr #16(w380) -> (w402:refnum<class "Engine Parent Editor Node.lvclass">, w401:errorcluster)
              n178 = call <vilib>:"read engine configuration.vi"("error in"=w401, "Engine Parent Editor Node in"=w402) -> ("error out"=w397:errorcluster, "engine configuration"=w398:refnum<class "engine configuration.lvclass">, "Engine Parent Editor Node out"=w400:refnum<class "Engine Parent Editor Node.lvclass">)  [unwired: 7 in]
              n179 = Unbundle By Name(w408) -> ("module configuration"=w407:refnum<class "alarms module configuration.lvclass">)
              n180 = call "check if alarm name exists.vi"("name to locate"=w406, "alarms module configuration in"=w407) -> ("alarm config"=w404:T12, "found?"=w405:bool)  [unwired: 6 in, 2 out]
              n181 = case shown="True" w405 {
                tunnel: w404 -> [_ w420]
                tunnel: w403 -> [_ w421]
                tunnel: w399 -> [_ w419]
                tunnel: w398 -> [_ w418]
                tunnel: [_ w415] -> w392
                frame False {
                }
                frame True {
                  n182 = case shown="1" w421 {
                    tunnel: w420 -> [_ w428 w430 w432]
                    tunnel: w419 -> [_ w426 _ _]
                    tunnel: [_ w424 w429 w431] -> w417
                    frame -1, Default {
                    }
                    frame 0 {
                      n183 = Unbundle By Name(w428) -> ("comparisons"=w427:T13[])
                      n184 = Index Array(array=w427, index=w426) -> (element=w425:T13)
                      n185 = Unbundle By Name(w425) -> ("input channel"=w424:refnum<class "TBM channel.lvclass">)
                    }
                    frame 1 {
                      n186 = Unbundle By Name(w430) -> ("unlatch"=w429:refnum<class "TBM channel.lvclass">)
                    }
                    frame 2 {
                      n187 = Unbundle By Name(w432) -> ("output"=w431:refnum<class "TBM channel.lvclass">)
                    }
                  }
                  n188 = call <vilib>:"filter tags available for mapping to channel.vi"("channel to map to"=w417, "engine configuration in"=w418) -> ("filtered tags"=w416:refnum<class "tag descriptor.lvclass">[])  [unwired: 8 in, 1 out]
                  n189 = for {
                    tunnel: w416 -> [w423] mode=indexing
                    tunnel: [w422] -> w415 mode=indexing
                    n190 = call <vilib>:"read tag name.vi"("system tag in"=w423) -> ("name"=w422:string)  [unwired: 8 in, 2 out]
                  }
                }
              }
              n191 = property class="CmbBox"(reference=w396) -> (reference out=w395:refnum<vi>, "Value"=w394:string)  [unwired: 1 in, 1 out]
              n192 = Search 1D Array(1D array=w392, element=w394) -> (index of element=w393:i32)  [unwired: 1 in]
              n193 = case shown="0.." w393 {
                selector: w393 -> [_ w414]
                tunnel: w392 -> [w409 w413]
                tunnel: [w409 w410] -> w391
                frame ..-1 {
                }
                frame 0.. {
                  n194 = Delete From Array(array=w413, index=w414) -> (deleted portion=w412:string, array with subset deleted=w411:string[])  [unwired: 1 in]
                  n195 = Build Array (concatenate)(w412, w411) -> (w410:string[])
                }
              }
              n196 = Build Array (concatenate)("", w391) -> (w389:string[])
              n197 = property class="CmbBox"(reference=w395, "Strings[]"=w389) -> ()  [unwired: 1 in, 2 out]
              n198 = in-place-dvr #15(w408) -> (w386:errorcluster)  [unwired: 1 out]
              n199 = in-place-dvr #16(w400) -> (w379:errorcluster)  [unwired: 1 out]
            }
            n200 = event-data("Discard?"=FALSE) -> ()  [unwired: 1 in, 1 out]
            n201 = Merge Errors(w377, w386, w379) -> (w385:errorcluster)
          }
          event "Add compare": Value Change {
            n202 = event-data() -> ()  [unwired: 1 in, 1 out]
            n203 = property on="Alarms" class="LstBox (strict)"() -> ("Item Names"=w436:string[], "Value"=w435:i32)  [unwired: 2 in, 2 out]
            n204 = Index Array(array=w436, index=w435) -> (element=w434:string)
            n205 = in-place {
              in-place-border: w434 -> [w449]
              in-place-border: [w447] -> w433
              n206 = in-place-dvr #17(w439) -> (w451:refnum<class "alarms module editor node.lvclass">, w441:errorcluster)
              n207 = control-ref of="Comparisons list"() -> (w448:refnum<vi>)
              n208 = Unbundle By Name(w451) -> ("module configuration"=w450:refnum<class "alarms module configuration.lvclass">)
              n209 = call "What shall we call this comparison?"("error in (no error)"=w441) -> ("Compare Name?"=w440:string, "OK"=w444:bool, "error out"=w443:errorcluster)  [unwired: 16 in]
              n210 = Compound Arithmetic op=AND(w444, invert w443) -> (w442:bool)
              n211 = case shown="True" w442 {
                tunnel: w450 -> [w452 w472]
                tunnel: w449 -> [_ w471]
                tunnel: w448 -> [_ w465]
                tunnel: w441 -> [w453 w459]
                tunnel: [w453 w458] -> w447
                tunnel: [w452 w455] -> w445
                tunnel: w440 -> [_ w454]
                frame False {
                }
                frame True {
                  n212 = property class="LstBox (strict)"(reference=w465) -> (reference out=w464:refnum<vi>, "Item Names"=w463:string[])  [unwired: 1 in, 1 out]
                  n213 = call "add alarm comparison.vi"("Limit"=inf, "comparison name"=w454, "comparison"=compare_type.">", "error in"=w459, "data type"=Data_Type."Double", "alarm name"=w471, "alarms module configuration in"=w472) -> ("error out"=w458:errorcluster, "created channels"=w467:refnum<class "TBM channel.lvclass">[], "compare index"=w460:i32, "alarms module configuration out"=w455:refnum<class "alarms module configuration.lvclass">)  [unwired: 1 in]
                  n214 = Index Array(array=w467) -> (element=w466:refnum<class "TBM channel.lvclass">)  [unwired: 1 in]
                  n215 = call <vilib>:"read tag name.vi"("system tag in"=w466) -> ("name"=w461:string)  [unwired: 8 in, 2 out]
                  n216 = Build Array (concatenate)(w463, w461) -> (w462:string[])
                  n217 = property class="LstBox (strict)"(reference=w464, "Item Names"=w462, "Val(Sgnl)"=w460) -> (error out=w456:errorcluster)  [unwired: 1 in, 1 out]
                  n218 = local read "Alarms"() -> (w457:i32)
                  n219 = property on="Alarms" class="LstBox (strict)"(error in=w456, "Val(Sgnl)"=w457) -> ()  [unwired: 1 in, 2 out]
                }
              }
              n220 = Bundle By Name(cluster=w451, "module configuration"=w445) -> (w446:refnum<class "alarms module editor node.lvclass">)
              n221 = in-place-dvr #17(w446) -> (w438:errorcluster)  [unwired: 1 out]
            }
            n222 = Merge Errors(w433, w438) -> (w437:errorcluster)
          }
          event "Remove compare": Value Change {
            n223 = event-data() -> ()  [unwired: 1 in, 1 out]
            n224 = property on="Alarms" class="LstBox (strict)"() -> ("Item Names"=w480:string[], "Value"=w479:i32)  [unwired: 2 in, 2 out]
            n225 = local read "Comparisons list"() -> (w474:i32)
            n226 = Index Array(array=w480, index=w479) -> (element=w478:string)
            n227 = in-place {
              in-place-border: w478 -> [w490]
              in-place-border: [w499] -> w475
              in-place-border: w474 -> [w489]
              in-place-border: [w486] -> w473
              n228 = in-place-dvr #18(w483) -> (w495:refnum<class "alarms module editor node.lvclass">)  [unwired: 1 out]
              n229 = in-place-dvr #19(w477) -> (w502:refnum<class "Engine Parent Editor Node.lvclass">, w501:errorcluster)
              n230 = control-ref of="Comparisons list"() -> ()  [unwired: 1 out]
              n231 = call <vilib>:"read engine configuration.vi"("error in"=w501, "Engine Parent Editor Node in"=w502) -> ("error out"=w500:errorcluster, "engine configuration"=w493:refnum<class "engine configuration.lvclass">, "Engine Parent Editor Node out"=w497:refnum<class "Engine Parent Editor Node.lvclass">)  [unwired: 7 in]
              n232 = Unbundle By Name(w495) -> ("module configuration"=w491:refnum<class "alarms module configuration.lvclass">)
              n233 = call <vilib>:"Read UID.vi"("configuration in"=w491) -> ("instance id"=w484:string, "configuration out"=w485:refnum<class "alarms module configuration.lvclass">)  [unwired: 8 in, 1 out]
              n234 = call "delete alarm comparison.vi"("compare index"=w489, "alarm name"=w490, "alarms module configuration in"=w485) -> ("error out"=w486:errorcluster, "removed channels"=w488:refnum<class "TBM channel.lvclass">[], "alarms module configuration out"=w487:refnum<class "alarms module configuration.lvclass">)  [unwired: 6 in]
              n235 = for {
                shift-right: [w505] -> w492
                shift-left: w493 -> [w506]
                tunnel: w488 -> [w504] mode=indexing
                tunnel: w484 -> [w503]
                n236 = call <vilib>:"delete mapping by channel.vi"("owner ID"=w503, "channel"=w504, "engine configuration in"=w506) -> ("engine configuration out"=w505:refnum<class "engine configuration.lvclass">)  [unwired: 7 in, 1 out]
              }
              n237 = local read "Alarms"() -> (w496:i32)
              n238 = property on="Alarms" class="LstBox (strict)"("Val(Sgnl)"=w496) -> ()  [unwired: 2 in, 2 out]
              n239 = Bundle By Name(cluster=w495, "module configuration"=w487) -> (w494:refnum<class "alarms module editor node.lvclass">)
              n240 = call <vilib>:"write engine configuration.vi"("error in"=w500, "engine configuration"=w492, "Engine Parent Editor Node in"=w497) -> ("error out"=w499:errorcluster, "Engine Parent Editor Node out"=w498:refnum<class "Engine Parent Editor Node.lvclass">)  [unwired: 7 in]
              n241 = in-place-dvr #18(w494) -> (w482:errorcluster)  [unwired: 1 out]
              n242 = in-place-dvr #19(w498) -> (w476:errorcluster)  [unwired: 1 out]
            }
            n243 = Merge Errors(w473, w475, w482, w476) -> (w481:errorcluster)
          }
          event "Output Tag", "Unlatch Tag", "Input Tag": Value Change {
            n244 = event-data() -> ("CtlRef"=w509:refnum<vi>, "NewVal"=w507:string)  [unwired: 1 in, 1 out]
            n245 = property on="Alarms" class="LstBox (strict)"() -> ("Item Names"=w517:string[], "Value"=w516:i32)  [unwired: 2 in, 2 out]
            n246 = local read "Comparisons list"() -> (w511:i32)
            n247 = Search 1D Array(1D array=w521, element=w509) -> (index of element=w514:i32)  [unwired: 1 in]
            n248 = Index Array(array=w517, index=w516) -> (element=w515:string)
            n249 = in-place {
              in-place-border: w515 -> [w541]
              in-place-border: w514 -> [w538]
              in-place-border: w511 -> [w535]
              in-place-border: [w534] -> w510
              in-place-border: w509 -> [_]
              in-place-border: [w530] -> w508
              in-place-border: w507 -> [w525]
              n250 = in-place-dvr #20(w520) -> (w542:refnum<class "alarms module editor node.lvclass">)  [unwired: 1 out]
              n251 = in-place-dvr #21(w513) -> (w537:refnum<class "Engine Parent Editor Node.lvclass">, w536:errorcluster)
              n252 = call <vilib>:"read engine configuration.vi"("error in"=w536, "Engine Parent Editor Node in"=w537) -> ("error out"=w533:errorcluster, "engine configuration"=w527:refnum<class "engine configuration.lvclass">, "Engine Parent Editor Node out"=w532:refnum<class "Engine Parent Editor Node.lvclass">)  [unwired: 7 in]
              n253 = Unbundle By Name(w542) -> ("module configuration"=w528:refnum<class "alarms module configuration.lvclass">)
              n254 = call "check if alarm name exists.vi"("name to locate"=w541, "alarms module configuration in"=w528) -> ("alarm config"=w539:T12, "found?"=w540:bool)  [unwired: 6 in, 2 out]
              n255 = call <vilib>:"Read UID.vi"("configuration in"=w528) -> ("instance id"=w523:string)  [unwired: 8 in, 2 out]
              n256 = case shown="True" w540 {
                tunnel: w539 -> [_ w556]
                tunnel: w538 -> [_ w557]
                tunnel: w535 -> [_ w555]
                tunnel: [_ w554] -> w522
                frame False {
                }
                frame True {
                  n257 = case shown="0" w557 {
                    tunnel: w556 -> [_ w563 w565 w567]
                    tunnel: w555 -> [_ w561 _ _]
                    tunnel: [_ w559 w564 w566] -> w554
                    frame -1, Default {
                    }
                    frame 0 {
                      n258 = Unbundle By Name(w563) -> ("comparisons"=w562:T13[])
                      n259 = local read "Alarms"() -> (w558:i32)
                      n260 = Index Array(array=w562, index=w561) -> (element=w560:T13)
                      n261 = property on="Alarms" class="LstBox (strict)"("Val(Sgnl)"=w558) -> ()  [unwired: 2 in, 2 out]
                      n262 = Unbundle By Name(w560) -> ("input channel"=w559:refnum<class "TBM channel.lvclass">)
                    }
                    frame 1 {
                      n263 = Unbundle By Name(w565) -> ("unlatch"=w564:refnum<class "TBM channel.lvclass">)
                    }
                    frame 2 {
                      n264 = Unbundle By Name(w567) -> ("output"=w566:refnum<class "TBM channel.lvclass">)
                    }
                  }
                }
              }
              n265 = call <vilib>:"delete mapping by channel.vi"("owner ID"=w523, "channel"=w522, "engine configuration in"=w527) -> ("error out"=w524:errorcluster, "engine configuration out"=w526:refnum<class "engine configuration.lvclass">)  [unwired: 7 in]
              n266 = call <vilib>:"Clear Errors.vi"("error in (no error)"=w524) -> ()  [unwired: 6 in, 1 out]
              n267 = case shown="Default" w525 {
                selector: w525 -> [w551 _]
                tunnel: [w545 _] -> w530
                tunnel: w526 -> [w552 w553]
                tunnel: [w546 w553] -> w529
                tunnel: w523 -> [w547 _]
                tunnel: w522 -> [w543 _]
                frame Default {
                  n268 = call <vilib>:"get full tag list.vi"("engine configuration in"=w552) -> ("tag list"=w549:refnum<class "tag descriptor.lvclass">[], "engine configuration out"=w548:refnum<class "engine configuration.lvclass">)  [unwired: 9 in]
                  n269 = call <vilib>:"find tag by name.vi"("name"=w551, "tags in"=w549) -> ("index"=w550:i32)  [unwired: 9 in]
                  n270 = Index Array(array=w549, index=w550) -> (element=w544:refnum<class "tag descriptor.lvclass">)
                  n271 = call <vilib>:"add mapping.vi"("owner ID"=w547, "channel"=w543, "tag descriptor"=w544, "engine configuration"=w548) -> ("error out"=w545:errorcluster, "engine configuration out"=w546:refnum<class "engine configuration.lvclass">)  [unwired: 6 in]
                }
                frame "" {
                }
              }
              n272 = call <vilib>:"write engine configuration.vi"("error in"=w533, "engine configuration"=w529, "Engine Parent Editor Node in"=w532) -> ("error out"=w534:errorcluster, "Engine Parent Editor Node out"=w531:refnum<class "Engine Parent Editor Node.lvclass">)  [unwired: 7 in]
              n273 = in-place-dvr #20(w542) -> (w519:errorcluster)  [unwired: 1 out]
              n274 = in-place-dvr #21(w531) -> (w512:errorcluster)  [unwired: 1 out]
            }
            n275 = Merge Errors(w508, w510, w519, w512) -> (w518:errorcluster)
          }
        }
        n276 = case shown="Error" w42 {
          selector: w42 -> [w51 w55]
          tunnel: [w52 w56] -> w48
          tunnel: w47 -> [w52 w56]
          tunnel: [w51 w53] -> w46
          frame No Error {
          }
          frame Error {
            # "#CodeRecommended Any errors should be handled within the generating case or here. Current default is to clear everything"
            n277 = call <vilib>:"Simple Error Handler.vi"("error in (no error)"=w55) -> ("error out"=w54:errorcluster)  [unwired: 4 in, 4 out]
            n278 = call <vilib>:"Clear Errors.vi"("error in (no error)"=w54) -> ("error out"=w53:errorcluster)  [unwired: 6 in]
          }
        }
      }
    }
    frame Error {
    }
  }
  n279 = Unregister For Events(event registration refnum=w24, error in=w23) -> (error out=w19:errorcluster)
  n280 = call <vilib>:"Simple Error Handler.vi"("error in (no error)"=w19) -> ()  [unwired: 4 in, 5 out]
